vi "RDV-addDataToGraph.vi"(8 "error in (no error)":errorcluster, 11 "RDV-Reflection_Data_viewer in":refnum<class "RDV-Reflection_Data_viewer.lvclass">) -> (0 "error out":errorcluster, 3 "RDV-Reflection_Data_viewer out":refnum<class "RDV-Reflection_Data_viewer.lvclass">)   [LabVIEW 2020, in "RDV-Reflection_Data_viewer.lvclass"]
doc: "Writes the data and the plot names of the viewer's map to its graphs."
uses:
  RDV-Reflection_Data_viewer.lvclass
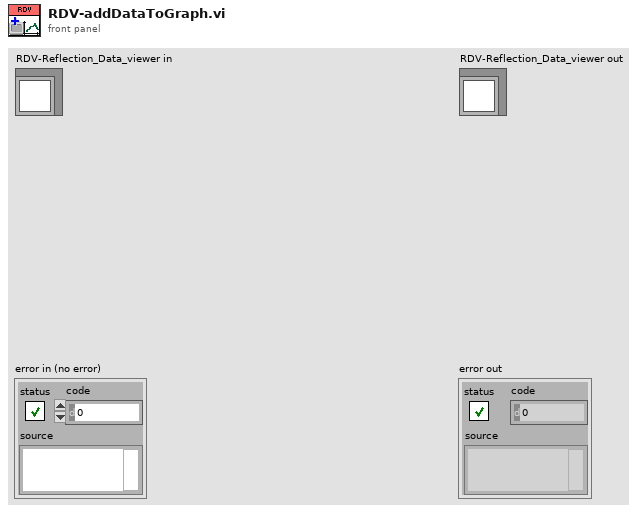
[diagram p1: front panel]
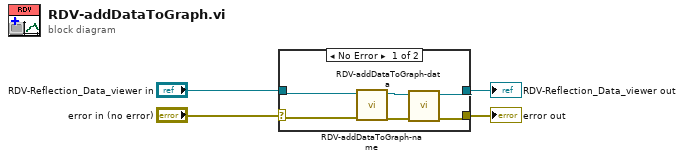
[diagram p0: block diagram]
diagram:
  n1 = case shown="No Error" "error in (no error)" {
    selector: "error in (no error)" -> [w5 w12]
    tunnel: [w7 w12] -> w3
    tunnel: [w9 w11] -> w1
    tunnel: "RDV-Reflection_Data_viewer in" -> [w8 w11]
    frame No Error {
      n2 = call "RDV-addDataToGraph-name.vi"("error in (no error)"=w5, "RDV-Reflection_Data_viewer in"=w8) -> ("error out"=w6:errorcluster, "RDV-Reflection_Data_viewer out"=w10:refnum<class "RDV-Reflection_Data_viewer.lvclass">)  [unwired: 8 in]
      n3 = call "RDV-addDataToGraph-data.vi"("error in (no error)"=w6, "RDV-Reflection_Data_viewer in"=w10) -> ("error out"=w7:errorcluster, "RDV-Reflection_Data_viewer out"=w9:refnum<class "RDV-Reflection_Data_viewer.lvclass">)  [unwired: 8 in]
    }
    frame Error {
    }
  }
  "error out" <- w3
  "RDV-Reflection_Data_viewer out" <- w1
